vi "PathPlanner_Trajectory_ReadCSVFile.vi"(8 "error in (no error)":errorcluster, 11 "FileName":string="trajectory.csv") -> (0 "error out":errorcluster, 3 "outTRAJECTORY":T1 {"States"."TargetHolonomicRotation"."SIN" format="%13.4f"; "States"."TargetHolonomicRotation"."COS" format="%13.4f"; "States"."TargetHolonomicRotation"."VALUE" format="%13.4f"; "States"."Heading"."SIN" format="%13.4f"; "States"."Heading"."COS" format="%13.4f"; "States"."Heading"."VALUE" format="%13.4f"; "States"."PositionMeters"."Y" format="%14.3f"; "States"."PositionMeters"."X" format="%14.3f"}, 4 "Full FIlename":string)   [LabVIEW 2019, in "PathPlanner24.lvlib"]
doc: "Create a trajectory from a CSV file. This can be used on a PC or the RoboRIO. Normally the CSV file is created as output from one of the trajectory utility programs. The file could also be created manually or by a custom written program.\n\nParameters:\n - FileName -- Name of the CSV file to read. See file name notes for additional information.\n - Error In -- Input error cluster (optional)\n\nReturns:\n - outTrajectory - Trajectory data structure cluster\n - Error out - returned error cluster\n\nNotes on use:\n -- This routine writes informational messges to the console and to the driver station log.\n\nNotes on file naming:\n -- The file name must include the extention. \".csv\" is not automatically appended to the name. \n -- The file name can be a simple file or an absolute path. If a simple file name is used the default path on the RoboRIO is: \"home:\\lvuser\\natinst\\LabVIEW Data\". On a Windows PC the default path is the LabVIEW default directory. Normally this is: “%HOMEDRIVE%%HOMEPATH%\\Documents\\LabView Data\".\n -- Filenames on the RoboRIO, which runs Linux, are case sensitive.\n\nNotes on file contents:\n -- Blank lines are ignored.\n -- Lines that begin with either #, !, or ' in the first character are considered comments and are ignored. \n -- Other lines are interpretted as comma separated data"
uses:
  PathPlanner24.lvlib
  TypeDef/PathPlannerTrajectory.ctl
  TypeDef/PathPlannerTrajectoryState.ctl
  <vilib>/Rock Robotics/WPI/ThirdParty/JAS_Junk/TrajLib/TypeDef/TRANSLATION2D.ctl
  <vilib>/Rock Robotics/WPI/ThirdParty/JAS_Junk/TrajLib/TypeDef/ROTATION2D.ctl
  TypeDef/PathPlannerPathConstraints.ctl
  <vilib>/Utility/error.llb/whitespace.ctl
  <vilib>/Rock Robotics/WPI/ThirdParty/JAS_Junk/TrajLib/Rotation2d_CreateAngle.vi
  <vilib>/Rock Robotics/WPI/ThirdParty/JAS_Junk/TrajLib/Util_CalcDist.vi
  <vilib>/Rock Robotics/WPI/ThirdParty/JAS_Junk/TrajLib/Trajectory_Library.lvlib
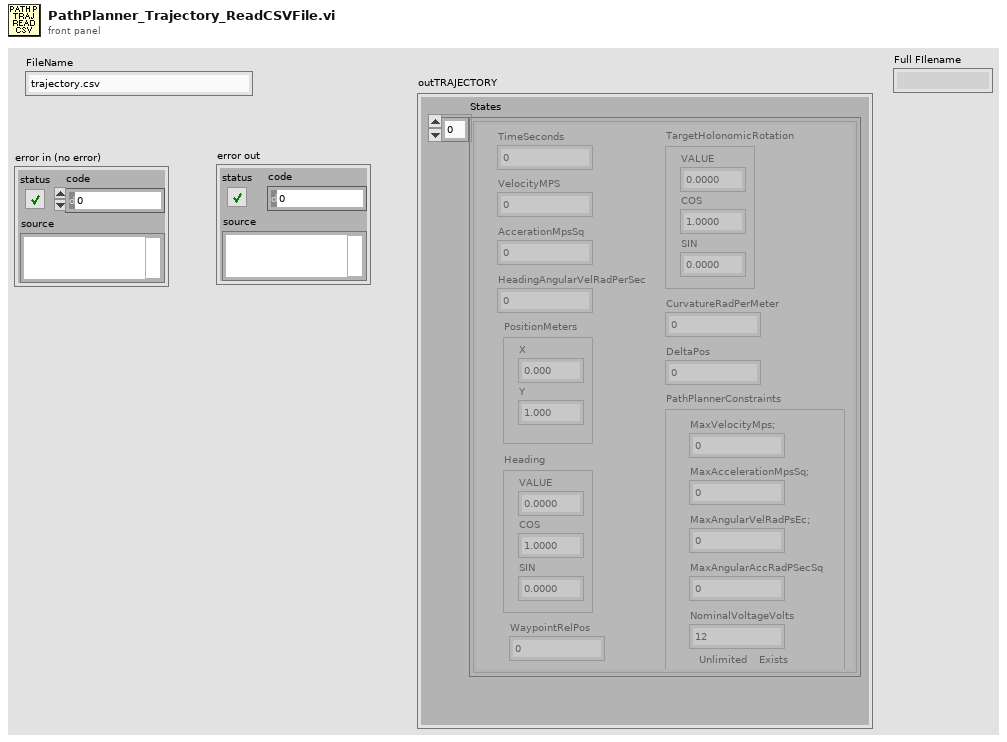
[diagram p1: front panel]
types:
  T1 = typedef "PathPlanner24.lvlib/PathPlannerTrajectory.ctl" = cluster{"States":T2[]}
  T2 = typedef "PathPlanner24.lvlib/PathPlannerTrajectoryState.ctl" = cluster{"TimeSeconds":dbl, "VelocityMPS":dbl, "AccerationMpsSq":dbl, "HeadingAngularVelRadPerSec":dbl, "PositionMeters":T3, "Heading":T4, "TargetHolonomicRotation":T4, "CurvatureRadPerMeter":dbl, "PathPlannerConstraints":T5, "DeltaPos":dbl, "WaypointRelPos":dbl}
  T3 = typedef "Trajectory_Library.lvlib/TRANSLATION2D.ctl" = cluster{"X":dbl, "Y":dbl}
  T4 = typedef "Trajectory_Library.lvlib/ROTATION2D.ctl" = cluster{"VALUE":dbl, "COS":dbl, "SIN":dbl}
  T5 = typedef "PathPlanner24.lvlib/PathPlannerPathConstraints.ctl" = cluster{"MaxVelocityMps;":dbl, "MaxAccelerationMpsSq;":dbl, "MaxAngularVelRadPsEc;":dbl, "MaxAngularAccRadPSecSq":dbl, "Exists":bool, "Unlimited":bool, "NominalVoltageVolts":dbl}
  T6 = enum16{"open", "replace", "create", "open or create", "replace or create", "replace or create with confirmation"}
  T7 = typedef "whitespace.ctl" = u16
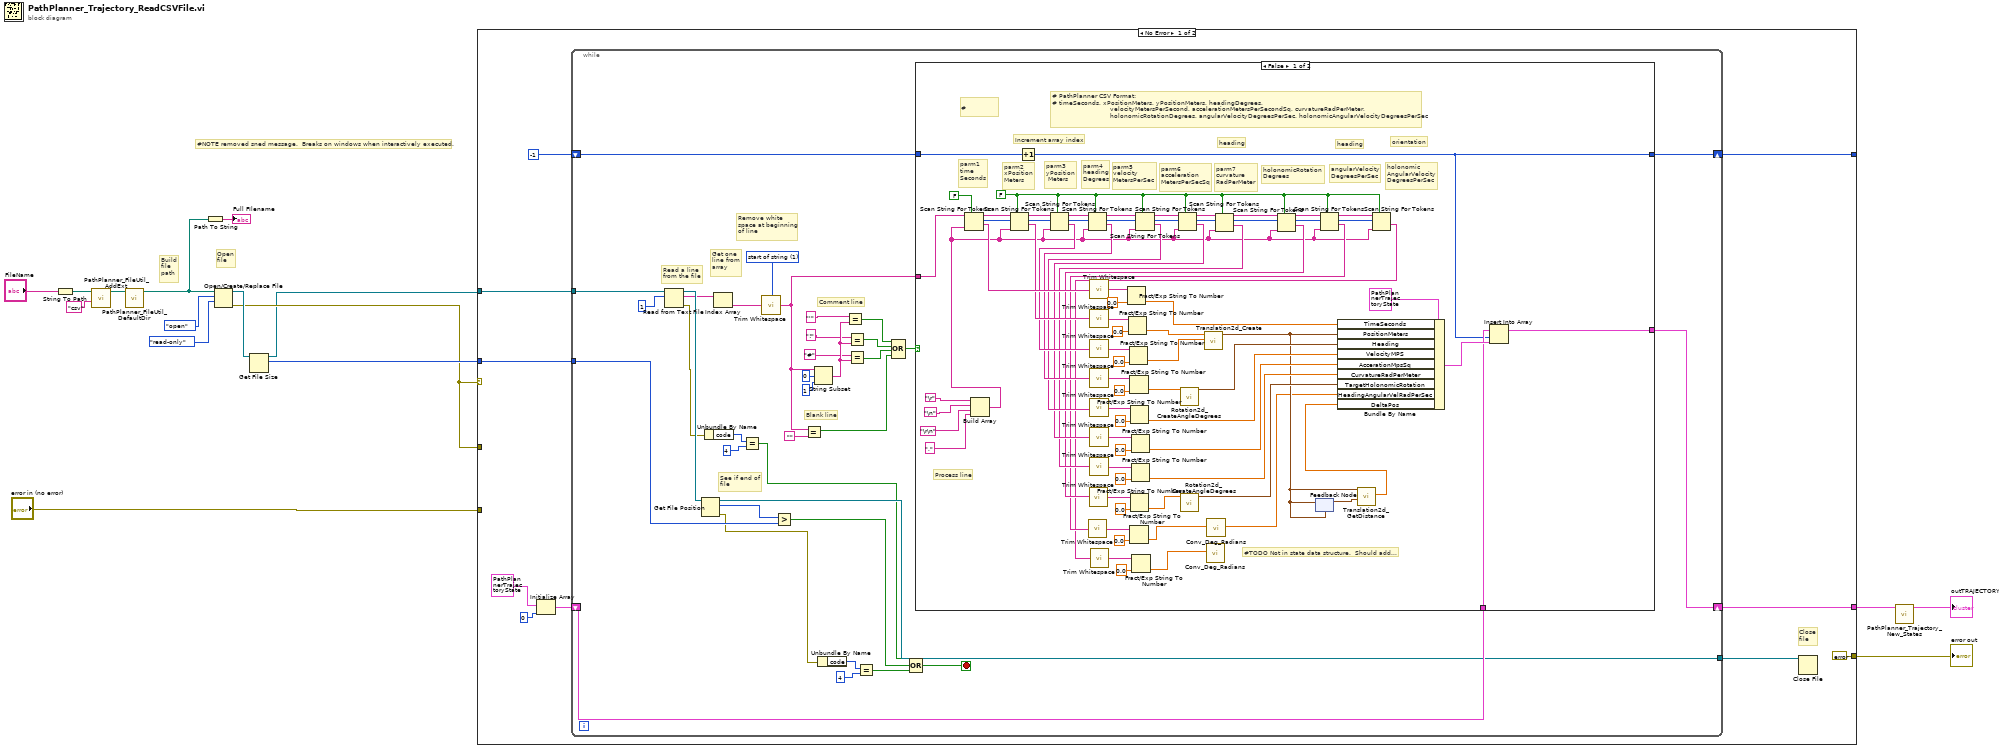
[diagram p0: block diagram]
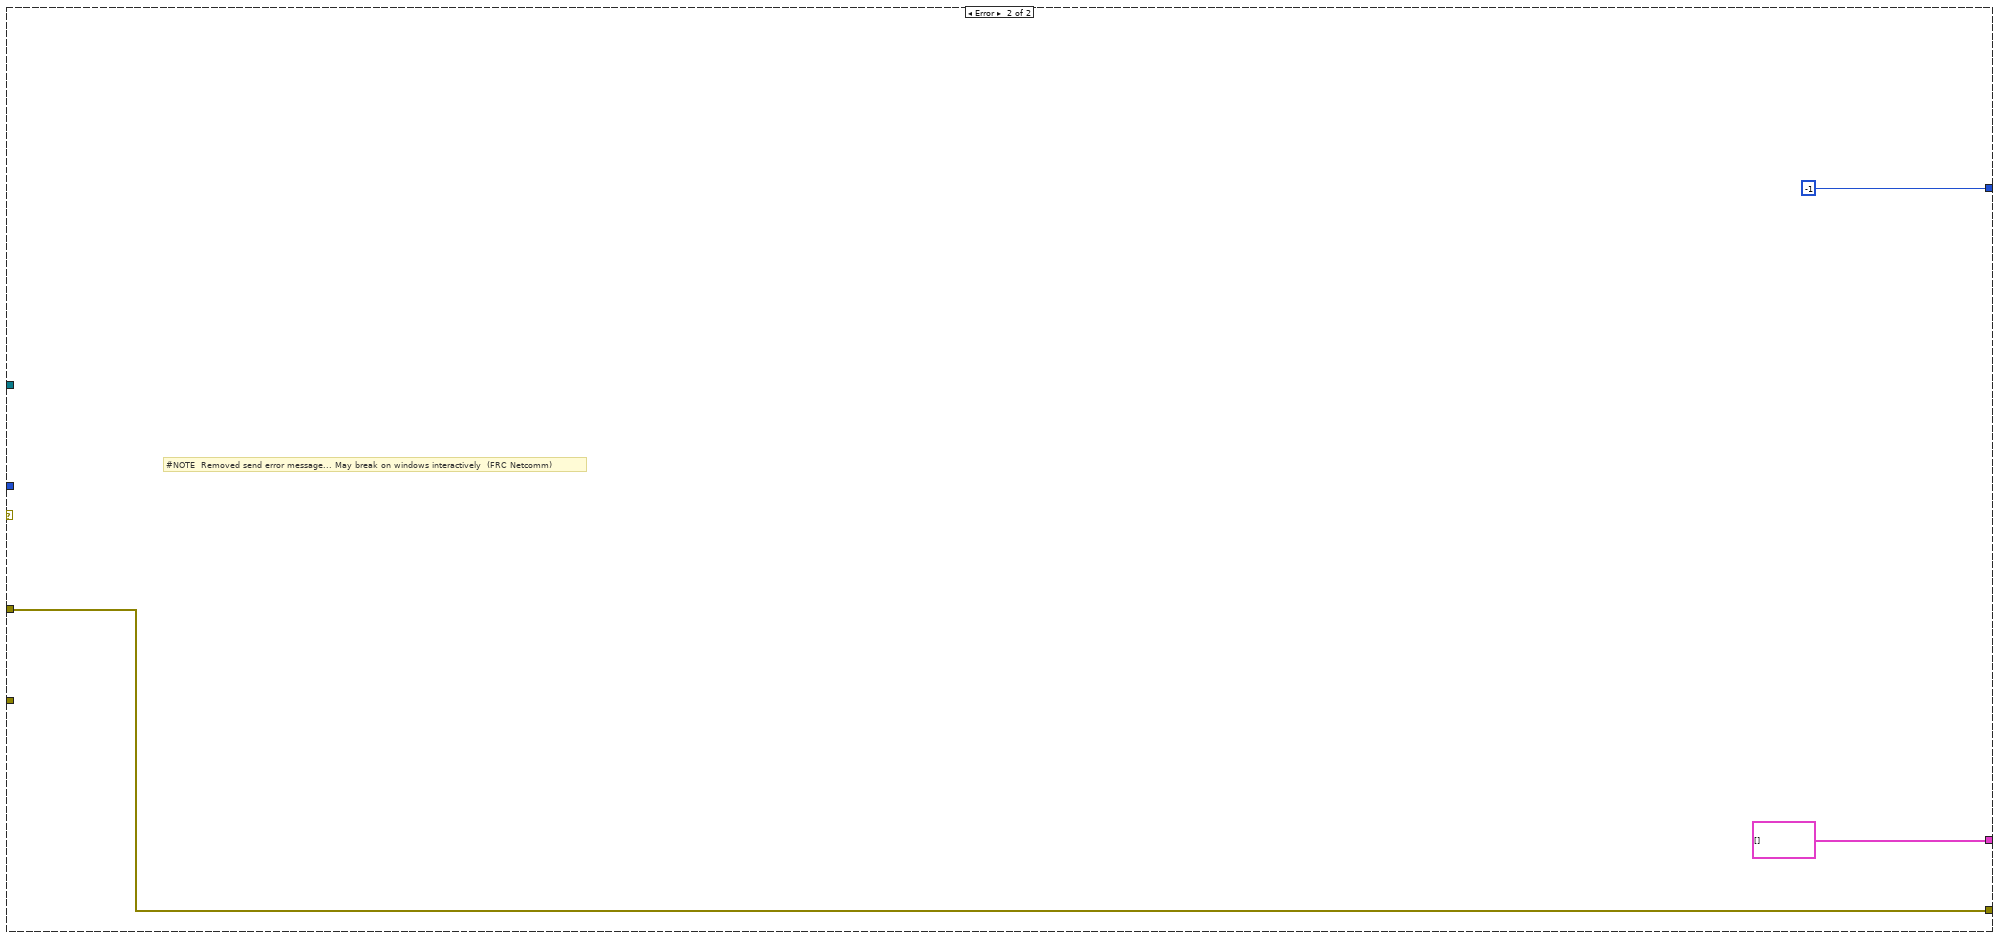
[diagram p3: hidden frame]
diagram:
  # "#NOTE removed sned message.  Breaks on windows when interactively executed."
  # "Open\nfile"
  # "Build\nfile\npath"
  n1 = String To Path(string="FileName") -> (path=w3:path)
  n2 = call "PathPlanner_FileUtil_AddExt.vi"("Extension"="csv", "Path in"=w3) -> ("Path out"=w4:path)  [unwired: 9 in]
  n3 = call "PathPlanner_FileUtil_DefaultDir.vi"("Path in"=w4) -> ("Path Out"=w2:path)  [unwired: 10 in]
  n4 = Path To String(path=w2) -> (string=→"Full FIlename":string)
  n5 = Open/Create/Replace File(file path (use dialog)=w2, operation (0:open)=T6."open", access (0:read/write)=enum16{"read/write", "read-only", "write-only"}."read-only") -> (refnum out=w14:refnum<file>, error out=w12:errorcluster)  [unwired: 3 in, 1 out]
  n6 = Get File Size(file=w14) -> (refnum out=w9:refnum<file>, size (in bytes)=w13:i64)  [unwired: 1 in, 1 out]
  n7 = case shown="No Error" w12 {
    tunnel: w9 -> [w26 _]
    tunnel: w13 -> [w24 _]
    tunnel: [w20 i16 -1] -> _
    tunnel: [w19 T2[] []] -> w6
    tunnel: w12 -> [_ w143]
    tunnel: [errorcluster {"status"=FALSE, "code"=0, "source"=""} ("error out") w143] -> w11
    tunnel: "error in (no error)" -> [_ _]
    frame No Error {
      # "Close\nfile"
      n8 = Initialize Array(T2 {"TimeSeconds"=0.0, "VelocityMPS"=0.0, "AccerationMpsSq"=0.0, "HeadingAngularVelRadPerSec"=0.0, "PositionMeters"={"X"=0.0, "Y"=1.0}, "Heading"={"VALUE"=0.0, "COS"=1.0, "SIN"=0.0}, "TargetHolonomicRotation"={"VALUE"=0.0, "COS"=1.0, "SIN"=0.0}, "CurvatureRadPerMeter"=0.0, "PathPlannerConstraints"={"MaxVelocityMps;"=0.0, "MaxAccelerationMpsSq;"=0.0, "MaxAngularVelRadPsEc;"=0.0, "MaxAngularAccRadPSecSq"=0.0, "Exists"=FALSE, "Unlimited"=FALSE, "NominalVoltageVolts"=12.0}, "DeltaPos"=0.0, "WaypointRelPos"=0.0} ("PathPlannerState"), 0 ("dimension size")) -> (w21:T2[])
      n9 = while {
        tunnel: w26 -> [w62]
        tunnel: w24 -> [w58]
        tunnel: [w38] -> w23
        shift-right: [w28] -> w20
        shift-left: i16 -1 -> [w42]
        shift-right: [w27] -> w19
        shift-left: w21 -> [w40]
        stop <- w36 stop-if-true
        w57 = T7 1 items=["both", "start of string", "end of string"] ("location (both)")
        # "Comment line"
        # "Blank line"
        # "Remove white \nspace at beginning\nof line"
        # "Get one\nline from\narray"
        # "Read a line\nfrom the file"
        # "See if end of \nfile"
        n10 = Read from Text File(file (use dialog)=w62, count=1) -> (refnum out=w60:refnum<file>, text=w56:string[], error out=w39:errorcluster)  [unwired: 2 in, 1 out]
        n11 = Get File Position(7:w60) -> (0:w31:errorcluster, 2:w59:i64, 3:w38:refnum<file>)  [unwired: 1 in]
        n12 = Unbundle By Name(w39) -> ("code"=w35:i32)
        n13 = Index Array(array=w56) -> (element=w55:string)  [unwired: 1 in]
        n14 = Equal?(x=w35, y=4) -> (x = y?=w30:bool)
        n15 = call <vilib>:"Trim Whitespace.vi"("string"=w55, "location (both)"=w57) -> ("trimmed string"=w41:string)
        n16 = Greater?(x=w59, y=w58) -> (0:w37:bool)
        n17 = Equal?(x=w41, y="") -> (x = y?=w44:bool)
        n18 = String Subset(string=w41, offset (0)=0, length (rest)=1 ("length (rest)")) -> (substring=w51:string)
        n19 = Unbundle By Name(w31) -> ("code"=w33:i32)
        n20 = Equal?(x="'", y=w51) -> (x = y?=w47:bool)
        n21 = Equal?(x="!", y=w51) -> (x = y?=w46:bool)
        n22 = Equal?(x="#", y=w51) -> (x = y?=w45:bool)
        n23 = Equal?(x=w33, y=4) -> (x = y?=w29:bool)
        n24 = Compound Arithmetic op=OR(w47, w46, w45, w44) -> (w43:bool)
        n25 = Compound Arithmetic op=OR(w30, w37, w29) -> (w36:bool)
        n26 = case shown="False" w43 {
          tunnel: w42 -> [w140 w141]
          tunnel: [w105 w141] -> w28
          tunnel: w41 -> [w104 _]
          tunnel: w40 -> [w107 w142]
          tunnel: [w106 w142] -> w27
          frame False {
            w91 = FALSE ("allow empty tokens? (F)")
            # "orientation"
            # "heading"
            # "heading"
            # "#TODO Not in state data structure.  Should add..."
            # "# PathPlanner CSV Format:\n# timeSeconds, xPositionMeters, yPositionMeters, headingDegrees, \n                             velocityMetersPerSecond, accelerationMetersPerSecondSq, curvatureRadPerMeter, \n                             holonomicRotationDegrees, angularVelocityDegreesPerSec, holonomicAngularVelocityDegreesPerSec"
            # "holonomic\nAngularVelocity\nDegreesPerSec"
            # "angularVelocity\nDegreesPerSec"
            # "holonomicRotation\nDegrees"
            # "#"
            # "parm6\nacceleration\nMetersPerSecSq"
            # "parm7\ncurvature\nRadPerMeter"
            # "parm5\nvelocity\nMetersPerSec"
            # "parm4\nheading\nDegrees"
            # "parm3\nyPosition\n Meters"
            # "parm2\nxPosition\nMeters"
            # "parm1\ntime\nSeconds"
            # "Increment array index"
            # "Process line"
            n27 = Build Array("\r", "\n", "\r\n", ",") -> (w74:string[])
            n28 = Scan String For Tokens(5:FALSE ("allow empty tokens? (F)"), 6:w74, 9:w104) -> (1:w124:string, 2:w129:i32, 3:w134:string)  [unwired: 3 in, 1 out]
            n29 = Scan String For Tokens(5:w91, 6:w74, 8:w129, 9:w134) -> (1:w123:string, 2:w128:i32, 3:w133:string)  [unwired: 2 in, 1 out]
            n30 = Increment(x=w140) -> (x+1=w105:i16)
            n31 = Scan String For Tokens(5:w91, 6:w74, 8:w128, 9:w133) -> (1:w122:string, 2:w127:i32, 3:w132:string)  [unwired: 2 in, 1 out]
            n32 = Scan String For Tokens(5:w91, 6:w74, 8:w127, 9:w132) -> (1:w121:string, 2:w126:i32, 3:w131:string)  [unwired: 2 in, 1 out]
            n33 = call <vilib>:"Trim Whitespace.vi"("string"=w124) -> ("trimmed string"=w96:string)  [unwired: 1 in]
            n34 = call <vilib>:"Trim Whitespace.vi"("string"=w123) -> ("trimmed string"=w117:string)  [unwired: 1 in]
            n35 = call <vilib>:"Trim Whitespace.vi"("string"=w122) -> ("trimmed string"=w112:string)  [unwired: 1 in]
            n36 = call <vilib>:"Trim Whitespace.vi"("string"=w121) -> ("trimmed string"=w111:string)  [unwired: 1 in]
            n37 = Fract/Exp String To Number(string=w96, default (0 dbl)=0.0 ("default (0 DBL)")) -> (number=w97:dbl)  [unwired: 2 in, 1 out]
            n38 = Fract/Exp String To Number(string=w117, default (0 dbl)=0.0 ("default (0 DBL)")) -> (number=w73:dbl)  [unwired: 2 in, 1 out]
            n39 = Fract/Exp String To Number(string=w112, default (0 dbl)=0.0 ("default (0 DBL)")) -> (number=w72:dbl)  [unwired: 2 in, 1 out]
            n40 = Fract/Exp String To Number(string=w111, default (0 dbl)=0.0 ("default (0 DBL)")) -> (number=w71:dbl)  [unwired: 2 in, 1 out]
            n41 = Scan String For Tokens(5:w91, 6:w74, 8:w126, 9:w131) -> (1:w120:string, 2:w125:i32, 3:w130:string)  [unwired: 2 in, 1 out]
            n42 = call <vilib>:"Trim Whitespace.vi"("string"=w120) -> ("trimmed string"=w110:string)  [unwired: 1 in]
            n43 = Fract/Exp String To Number(string=w110, default (0 dbl)=0.0 ("default (0 DBL)")) -> (number=w94:dbl)  [unwired: 2 in, 1 out]
            n44 = Scan String For Tokens(5:w91, 6:w74, 8:w125, 9:w130) -> (1:w119:string, 2:w99:i32, 3:w100:string)  [unwired: 2 in, 1 out]
            n45 = call <vilib>:"Trim Whitespace.vi"("string"=w119) -> ("trimmed string"=w109:string)  [unwired: 1 in]
            n46 = Fract/Exp String To Number(string=w109, default (0 dbl)=0.0 ("default (0 DBL)")) -> (number=w93:dbl)  [unwired: 2 in, 1 out]
            n47 = call <vilib>:"Rotation2d_CreateAngleDegrees.vi"("Angle_Degrees"=w71) -> ("ROTATION"=w70:T4)  [unwired: 10 in]
            n48 = call <vilib>:"Translation2d_Create.vi"("Y"=w72, "X"=w73) -> ("TRANSLATION"=w66:T3)  [unwired: 9 in]
            n49 = Scan String For Tokens(5:w91, 6:w74, 8:w99, 9:w100) -> (1:w98:string, 2:w87:i32, 3:w90:string)  [unwired: 2 in, 1 out]
            n50 = call <vilib>:"Trim Whitespace.vi"("string"=w98) -> ("trimmed string"=w101:string)  [unwired: 1 in]
            n51 = Fract/Exp String To Number(string=w101, default (0 dbl)=0.0 ("default (0 DBL)")) -> (number=w92:dbl)  [unwired: 2 in, 1 out]
            n52 = Scan String For Tokens(5:w91, 6:w74, 8:w87, 9:w90) -> (1:w78:string, 2:w86:i32, 3:w89:string)  [unwired: 2 in, 1 out]
            n53 = call <vilib>:"Trim Whitespace.vi"("string"=w78) -> ("trimmed string"=w83:string)  [unwired: 1 in]
            n54 = Fract/Exp String To Number(string=w83, default (0 dbl)=0.0 ("default (0 DBL)")) -> (number=w77:dbl)  [unwired: 2 in, 1 out]
            n55 = call <vilib>:"Rotation2d_CreateAngleDegrees.vi"("Angle_Degrees"=w77) -> ("ROTATION"=w69:T4)  [unwired: 10 in]
            n56 = feedback-in #1(w66) -> ()
            n57 = feedback #1(w66) -> (w65:T3)
            n58 = Scan String For Tokens(5:w91, 6:w74, 8:w86, 9:w89) -> (1:w76:string, 2:w85:i32, 3:w88:string)  [unwired: 2 in, 1 out]
            n59 = call <vilib>:"Trim Whitespace.vi"("string"=w76) -> ("trimmed string"=w81:string)  [unwired: 1 in]
            n60 = Fract/Exp String To Number(string=w81, default (0 dbl)=0.0 ("default (0 DBL)")) -> (number=w68:dbl)  [unwired: 2 in, 1 out]
            n61 = call <vilib>:"Conv_Deg_Radians.vi"("Degress"=w68) -> ("Radians"=w63:dbl)  [unwired: 10 in]
            n62 = call <vilib>:"Translation2d_GetDistance.vi"("other Translation"=w65, "In Translation"=w66) -> ("Distance"=w64:dbl)  [unwired: 9 in]
            n63 = Bundle By Name(cluster=T2 {"TimeSeconds"=0.0, "VelocityMPS"=0.0, "AccerationMpsSq"=0.0, "HeadingAngularVelRadPerSec"=0.0, "PositionMeters"={"X"=0.0, "Y"=1.0}, "Heading"={"VALUE"=0.0, "COS"=1.0, "SIN"=0.0}, "TargetHolonomicRotation"={"VALUE"=0.0, "COS"=1.0, "SIN"=0.0}, "CurvatureRadPerMeter"=0.0, "PathPlannerConstraints"={"MaxVelocityMps;"=0.0, "MaxAccelerationMpsSq;"=0.0, "MaxAngularVelRadPsEc;"=0.0, "MaxAngularAccRadPSecSq"=0.0, "Exists"=FALSE, "Unlimited"=FALSE, "NominalVoltageVolts"=12.0}, "DeltaPos"=0.0, "WaypointRelPos"=0.0} ("PathPlannerState"), "TimeSeconds"=w97, "PositionMeters"=w66, "Heading"=w70, "VelocityMPS"=w94, "AccerationMpsSq"=w93, "CurvatureRadPerMeter"=w92, "TargetHolonomicRotation"=w69, "HeadingAngularVelRadPerSec"=w63, "DeltaPos"=w64) -> (w108:T2)
            n64 = Scan String For Tokens(5:w91, 6:w74, 8:w85, 9:w88) -> (1:w75:string)  [unwired: 2 in, 3 out]
            n65 = call <vilib>:"Trim Whitespace.vi"("string"=w75) -> ("trimmed string"=w79:string)  [unwired: 1 in]
            n66 = Fract/Exp String To Number(string=w79, default (0 dbl)=0.0 ("default (0 DBL)")) -> (number=w67:dbl)  [unwired: 2 in, 1 out]
            n67 = call <vilib>:"Conv_Deg_Radians.vi"("Degress"=w67) -> ()  [unwired: 10 in, 1 out]
            n68 = Insert Into Array(array=w107, index=w105, new element=w108) -> (w106:T2[])
          }
          frame True {
            # "Comment -- ignore."
          }
        }
      }
      n69 = Close File(refnum=w23) -> ()  [unwired: 1 in, 2 out]
    }
    frame Error {
      # "#NOTE  Removed send error message... May break on windows interactively  (FRC Netcomm)"
    }
  }
  "error out" <- w11
  n70 = call "PathPlanner_Trajectory_New_States.vi"("PathPlannerStates"=w6) -> ("PathPlannerTrajectory"=→"outTRAJECTORY":T1)  [unwired: 10 in]
